vi "ROI entry-Event handler-Clear All ROI.vi"   [LabVIEW 2020]
uses:
  Typedefs/ROI management FG states.ctl
  Typedefs/FGV ROI Time Ops.ctl
types:
  T1 = typedef "FGV ROI Time Ops.ctl" = enum16{"Read", "Write Cycle Time", "Write Cycle Rate"}
  T2 = typedef "ROI management FG states.ctl" = enum16{"Read", "Write", "Write-from dataset", "Clear Last", "Clear All", "Delete ROI", "Update ROIs time", "Reload last ROI set", "Modify ROI Parameters", "Offset all ROI", "Offset visible ROI", "Modify Dwell Time", "Modify Laser Power"}
  T3 = typedef "ROI ID Enum.ctl" = enum16{"Point", "MiniScan", "Comp. MiniScan", "Rectangle", "Comp. volume", "Arb. plane point", "None"}
  T4 = typedef "ROI parameters data type.ctl" = cluster{"ROI index":dbl, "ROI ID":dbl, "ROI Time (ns)":dbl, "Pixels in ROI":dbl, "X start":dbl, "Y start":dbl, "Z start":dbl, "X stop":dbl, "Y stop":dbl, "Z stop":dbl, "Angle (deg)":dbl, "Composite ID":dbl, "Number of lines":dbl, "Frame Size":dbl, "Zoom":dbl, "Laser Power (%)":dbl, "ROI group ID":dbl, "Resolution":dbl, "Dwell Time per pixel":dbl, "Pixels per miniscan":dbl, "Original FOV (um)":dbl, "Apparent Frame Size":dbl, "Z Plane Idx":i32[], "Z Plane codes":i32[]}
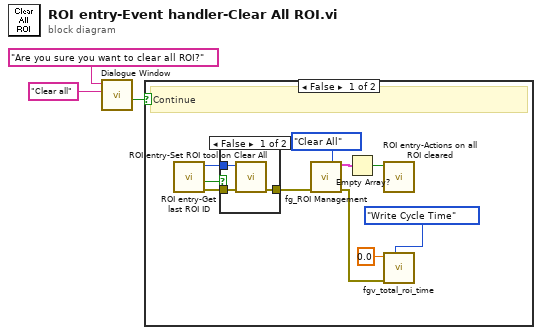
[diagram p0: block diagram]
diagram:
  n1 = call "Dialogue Window.vi"("Caption-Right button (OK)"="Clear all" ("T button name (\"OK\")"), "Message string"="Are you sure you want to clear all ROI?" ("message")) -> ("Cancelled (Left button pressed)"=w3:bool)  [unwired: 7 in, 2 out]
  n2 = case shown="False" w3 {
    frame False {
      # "Continue"
      n3 = call "ROI entry-Get last ROI ID.vi"() -> ("error out"=w8:errorcluster, "NO ROI"=w7:bool, "ROI ID Enum"=w9:T3)  [unwired: 8 in, 1 out]
      n4 = case shown="False" w7 {
        tunnel: [w16 w17] -> w10
        tunnel: w9 -> [w15 _]
        tunnel: w8 -> [w14 w17]
        frame False {
          n5 = call "ROI entry-Set ROI tool on Clear All.vi"("error in (no error)"=w14, "Last ROI ID Enum"=w15) -> ("error out"=w16:errorcluster)  [unwired: 9 in]
        }
        frame True {
        }
      }
      n6 = call "fg_ROI Management.vi"("Function"=ROI_management_FG_states."Clear All", "error in (no error)"=w10) -> ("ROI Setup"=w12:T4[], "error out"=w6:errorcluster)  [unwired: 7 in, 5 out]
      n7 = Empty Array?(array=w12) -> (empty?=w13:bool)
      n8 = call "ROI entry-Actions on all ROI cleared.vi"("No ROIs (T)"=w13) -> ()  [unwired: 11 in]
      n9 = call "fgv_total_roi_time.vi"("Op"=FGV_ROI_Time_Ops."Write Cycle Time", "error in (no error)"=w6, "Total cycle time"=0.0) -> ()  [unwired: 4 in, 5 out]
    }
    frame True {
      # "Cancelled"
    }
  }
